vi "PathPlanner_PathFinder_FindClosestNonObstacle.vi"(11 "GridPosition":T1) -> (1 "Found":bool, 3 "NonObstacleGridPositin":T1)   [LabVIEW 2019, in "PathPlanner24.lvlib"]
doc: "Internal function. Not to be used by end users."
uses:
  PathPlanner24.lvlib
  TypeDef/PathPlannerFinderGridPosition.ctl
  PathPlanner_GridPosition_Get.vi
  PathPlanner_GridPosition_New.vi
  PathPlanner_PathFinder_Globals.vi
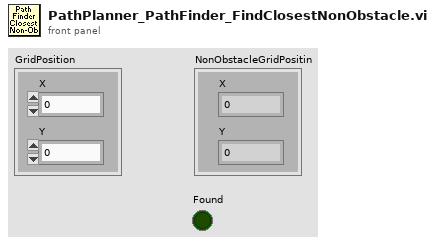
[diagram p1: front panel]
types:
  T1 = typedef "PathPlanner24.lvlib/PathPlannerFinderGridPosition.ctl" = cluster{"X":i32, "Y":i32}
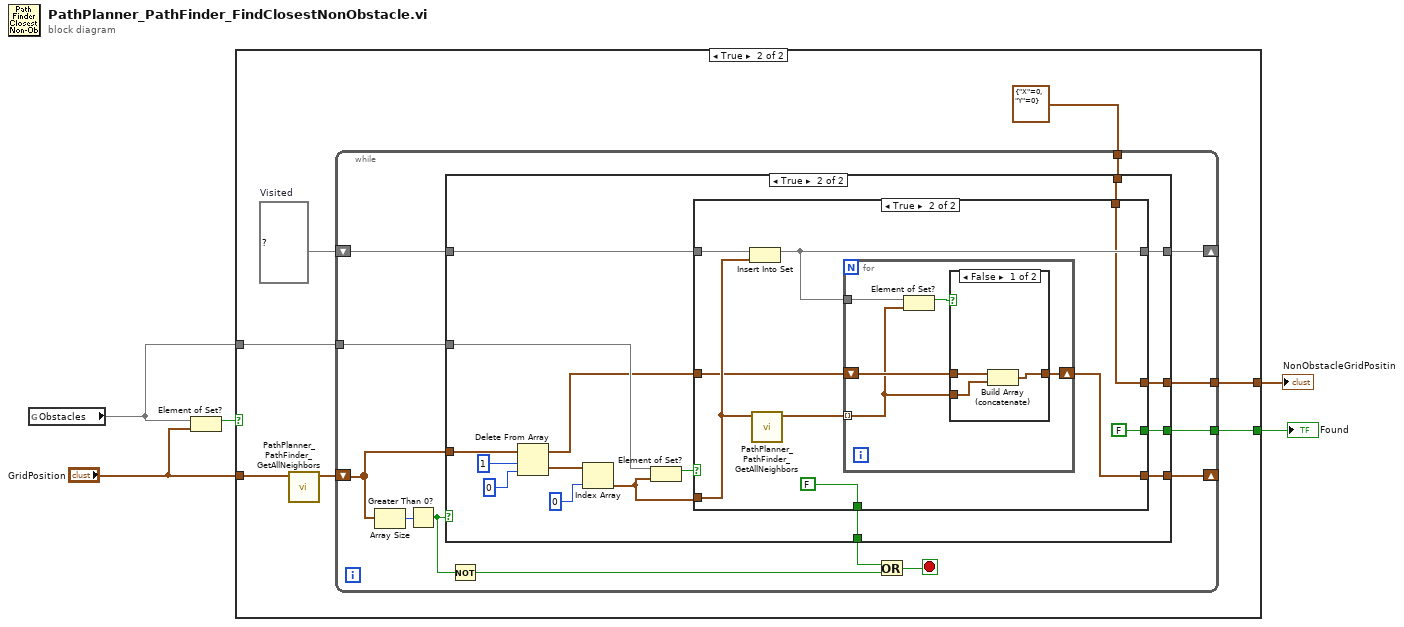
[diagram p0: block diagram]
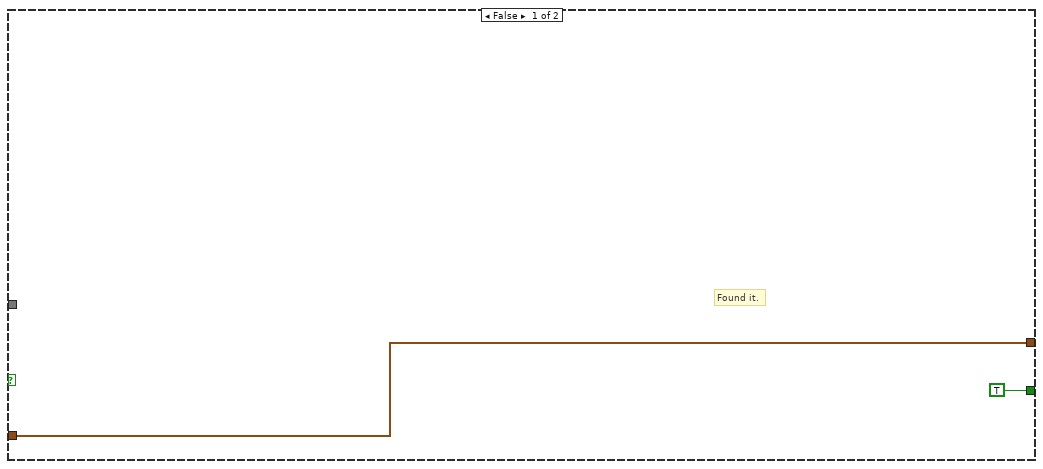
[diagram p2: hidden frame]
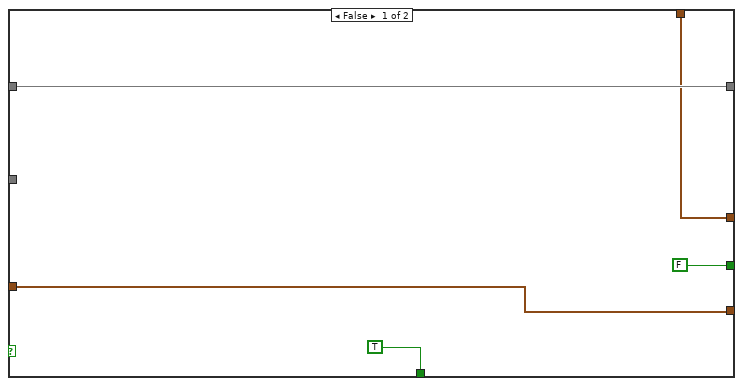
[diagram p3: hidden frame]
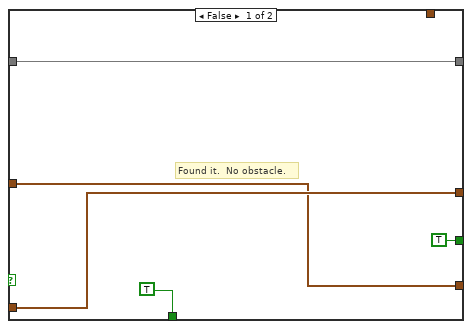
[diagram p4: hidden frame]
diagram:
  n1 = global read "PathPlanner_PathFinder_Globals.vi" "Obstacles"() -> (w2:set{T1})
  n2 = Element of Set?(10:"GridPosition", 11:w2) -> (3:w5:bool)
  n3 = case shown="True" w5 {
    tunnel: "GridPosition" -> [w7 w14]
    tunnel: [w7 w11] -> w3
    tunnel: w2 -> [_ w12]
    tunnel: [TRUE ("Found") w9] -> w1
    frame False {
      # "Found it."
    }
    frame True {
      w10 = set{T1} {}  # Visited
      n4 = call "PathPlanner_PathFinder_GetAllNeighbors.vi"("GridPosition"=w14) -> ("Neighbors"=w13:T1[])  [unwired: 10 in]
      n5 = while {
        shift-right: [w17] -> _
        shift-left: w13 -> [w22]
        tunnel: w12 -> [w21]
        tunnel: [w20] -> w11
        shift-right: [w18] -> _
        shift-left: w10 -> [w19]
        tunnel: [w16] -> w9
        tunnel: T1 {"X"=0, "Y"=0} ("Neighbors") -> [w15]
        stop <- w25 stop-if-true
        n6 = Array Size(array=w22) -> (size(s)=w27:i32)
        n7 = Greater Than 0?(x=w27) -> (x > 0?=w26:bool)
        n8 = case shown="True" w26 {
          tunnel: [TRUE w43] -> w23
          tunnel: w22 -> [w29 w39]
          tunnel: w21 -> [_ w45]
          tunnel: [w28 w42] -> w20
          tunnel: w19 -> [w31 w40]
          tunnel: [w31 w38] -> w18
          tunnel: [w29 w37] -> w17
          tunnel: [FALSE w36] -> w16
          tunnel: w15 -> [w28 w35]
          frame False {
          }
          frame True {
            n9 = Delete From Array(array=w39, length=1, index=0) -> (deleted portion=w34:T1[], array with subset deleted=w33:T1[])
            n10 = Index Array(array=w34, index=0) -> (element=w41:T1)
            n11 = Element of Set?(10:w41, 11:w45) -> (3:w44:bool)
            n12 = case shown="True" w44 {
              tunnel: [TRUE FALSE] -> w43
              tunnel: [w52 w54] -> w42
              tunnel: w41 -> [w52 w60]
              tunnel: w40 -> [w50 w61]
              tunnel: w33 -> [w51 w58]
              tunnel: [w50 w57] -> w38
              tunnel: [w51 w56] -> w37
              tunnel: [TRUE FALSE] -> w36
              tunnel: w35 -> [_ w54]
              frame False {
                # "Found it.  No obstacle."
              }
              frame True {
                n13 = Insert Into Set(10:w60, 11:w61) -> (3:w57:set{T1})  [unwired: 1 out]
                n14 = call "PathPlanner_PathFinder_GetAllNeighbors.vi"("GridPosition"=w60) -> ("Neighbors"=w59:T1[])  [unwired: 10 in]
                n15 = for {
                  tunnel: w59 -> [w63] mode=indexing
                  shift-right: [w64] -> w56
                  shift-left: w58 -> [w65]
                  tunnel: w57 -> [w67]
                  n16 = Element of Set?(10:w63, 11:w67) -> (3:w66:bool)
                  n17 = case shown="False" w66 {
                    tunnel: w65 -> [w70 w71]
                    tunnel: [w68 w71] -> w64
                    tunnel: w63 -> [w69 _]
                    frame False {
                      n18 = Build Array (concatenate)(w70, w69) -> (w68:T1[])
                    }
                    frame True {
                    }
                  }
                }
              }
            }
          }
        }
        n19 = Not(x=w26) -> (.not. x?=w24:bool)
        n20 = Or(x=w23, y=w24) -> (x .or. y?=w25:bool)
      }
    }
  }
  "NonObstacleGridPositin" <- w3
  "Found" <- w1
